vi "Initialize.vi"(8 "error in (no error)":errorcluster, 10 "Info":T1, 11 "Image in":refnum<class "SVGImage.lvclass">) -> (0 "error out":errorcluster, 3 "Image out":refnum<class "SVGImage.lvclass">)   [LabVIEW 2019, in "SVGImage.lvclass"]
uses:
  SVGImage.lvclass
  C:/Users/Albro/Documents/GitHub/AFM-Lithography/lvsrc/Classes/Parse/SVG Object/SVG Object.lvclass
  InitializationInfo.ctl
  TransformTokenizer/TransformTokenizer.lvclass
  TransformTokenizer/TransformTokenizer.lvclass/TransformTokenizer.ctl
  SVGImage.lvclass/SVGImage.ctl
  Transform/Transform.lvclass
  Transform.Matrix/Transform.Matrix.lvclass
  C:/Users/Albro/Documents/GitHub/AFM-Lithography/lvsrc/Classes/Parse/Transform/Transform.lvclass
  Transform.Translate/Transform.Translate.lvclass
  Transform.Rotate/Transform.Rotate.lvclass
  Transform.Skew/Transform.Skew.lvclass
  PathCommands/Point.ctl
  Transform/Transform.lvclass/Transform.ctl
  <vilib>/Analysis/baseanly.llb/Real A x B.vi
  Write X.vi
  Write Y.vi
  Write Width.vi
  Write Height.vi
  Write Path.vi
  Read Width.vi
  Read X.vi
  Read Height.vi
  Read Y.vi
  <vilib>/LabVIEW Open Source Project/OpenURI/openURI.lvlib
  PathCommands/PathCommands.lvclass
  <vilib>/Analysis/NI_AALBase.lvlib
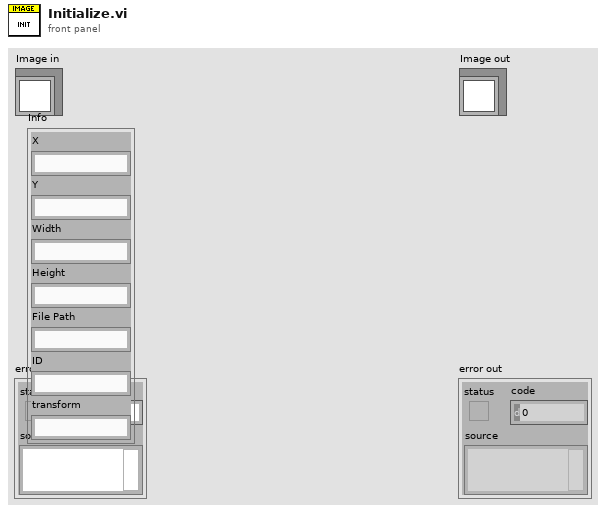
[diagram p1: front panel]
types:
  T1 = typedef "SVGImage.lvclass/InitializationInfo.ctl" = cluster{"X":string, "Y":string, "Width":string, "Height":string, "File Path":string, "ID":string, "transform":string}
  T2 = typedef "PathCommands.lvclass/Point.ctl" = cluster{"X":dbl, "Y":dbl}
  T3 = typedef "NI_Matrix.lvlib/RealMatrix.ctl" = dbl[][]
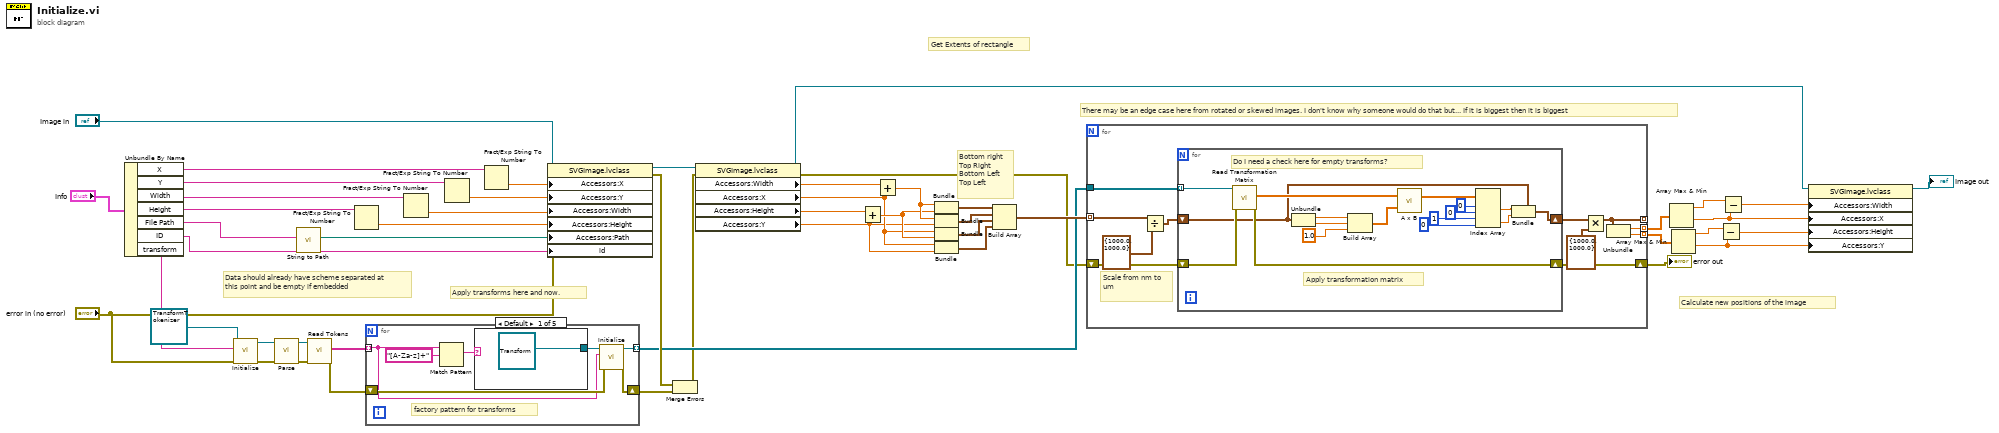
[diagram p0: block diagram]
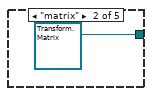
[diagram p2: hidden frame]
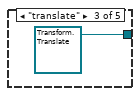
[diagram p3: hidden frame]
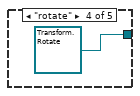
[diagram p4: hidden frame]
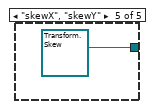
[diagram p5: hidden frame]
diagram:
  # "There may be an edge case here from rotated or skewed images. I don't know why someone would do that but... If it is biggest then it is biggest"
  # "Calculate new positions of the image"
  # "Get Extents of rectangle"
  # "Bottom right\nTop Right\nBottom Left\nTop Left"
  # "Apply transforms here and now."
  # "Data should already have scheme separated at this point and be empty if embedded"
  n1 = Unbundle By Name("Info") -> ("X"=w48:string, "Y"=w47:string, "Width"=w46:string, "Height"=w45:string, "File Path"=w39:string, "ID"=w38:string, "transform"=w1:string)
  n2 = call "Initialize.vi"("error in (no error)"="error in (no error)", "Transform Attribute String"=w1, "TransformTokenizer in"=refnum<class "TransformTokenizer.lvclass"> refnum) -> ("error out"=w37:errorcluster, "TransformTokenizer out"=w33:refnum<class "TransformTokenizer.lvclass">)  [unwired: 7 in]
  n3 = call "Parse.vi"("error in (no error)"=w37, "TransformTokenizer in"=w33) -> ("error out"=w36:errorcluster, "TransformTokenizer out"=w31:refnum<class "TransformTokenizer.lvclass">)  [unwired: 8 in]
  n4 = call <vilib>:"String to Path.vi"("common path"=w39) -> ("Path"=w40:path)  [unwired: 10 in]
  n5 = call "Read Tokens.vi"("error in (no error)"=w36, "TransformTokenizer in"=w31) -> ("error out"=w35:errorcluster, "Transforms"=w30:string[])  [unwired: 7 in, 1 out]
  n6 = Fract/Exp String To Number(string=w45) -> (number=w41:dbl)  [unwired: 3 in, 1 out]
  n7 = for {
    tunnel: w30 -> [w51] mode=indexing
    shift-right: [w53] -> w34
    shift-left: w35 -> [w54]
    tunnel: [w52] -> w15 mode=indexing
    # "factory pattern for transforms"
    n8 = Match Pattern(string=w51, regular expression="[A-Za-z]+") -> (match substring=w56:string)  [unwired: 1 in, 3 out]
    n9 = case shown="Default" w56 {
      tunnel: [refnum<class "Transform.lvclass"> refnum ("Transform in") refnum<class "Transform.Matrix.lvclass"> refnum ("Transform.Matrix.lvclass") refnum<class "Transform.Translate.lvclass"> refnum ("Transform.Translate.lvclass") refnum<class "Transform.Rotate.lvclass"> refnum ("Transform.Rotate.lvclass") refnum<class "Transform.Skew.lvclass"> refnum ("Transform.Skew.lvclass")] -> w55
      frame Default {
      }
      frame "matrix" {
      }
      frame "translate" {
      }
      frame "rotate" {
      }
      frame "skewX", "skewY" {
      }
    }
    n10 = call-dynamic "Initialize.vi"("error in (no error)"=w54, "Transform"=w51, "Transform in"=w55) -> ("error out"=w53:errorcluster, "Transform out"=w52:refnum<class "Transform.lvclass">)  [unwired: 7 in]
  }
  n11 = Fract/Exp String To Number(string=w46) -> (number=w42:dbl)  [unwired: 3 in, 1 out]
  n12 = Fract/Exp String To Number(string=w47) -> (number=w43:dbl)  [unwired: 3 in, 1 out]
  n13 = Fract/Exp String To Number(string=w48) -> (number=w44:dbl)  [unwired: 3 in, 1 out]
  n14 = property class="SVGImage.lvclass"(reference="Image in", error in="error in (no error)", "Accessors:X"=w44, "Accessors:Y"=w43, "Accessors:Width"=w42, "Accessors:Height"=w41, "Accessors:Path"=w40, "id"=w38) -> (reference out=w21:refnum<class "SVGImage.lvclass">, error out=w16:errorcluster)
  n15 = Merge Errors(w16, w34) -> (w13:errorcluster)
  n16 = property class="SVGImage.lvclass"(reference=w21, error in=w13) -> (reference out=w10:refnum<class "SVGImage.lvclass">, error out=w12:errorcluster, "Accessors:Width"=w20:dbl, "Accessors:X"=w19:dbl, "Accessors:Height"=w18:dbl, "Accessors:Y"=w17:dbl)
  n17 = Add(x=w18, y=w17) -> (x+y=w27:dbl)
  n18 = Add(x=w20, y=w19) -> (x+y=w28:dbl)
  n19 = Bundle(w28, w27) -> (w26:cluster{dbl, dbl})  [unwired: 1 in]
  n20 = Bundle(w28, "Accessors:Y"=w17) -> (w23:cluster{dbl, "Accessors:Y":dbl})  [unwired: 1 in]
  n21 = Bundle("Accessors:X"=w19, w27) -> (w25:cluster{"Accessors:X":dbl, dbl})  [unwired: 1 in]
  n22 = Bundle("Accessors:X"=w19, "Accessors:Y"=w17) -> (w24:cluster{"Accessors:X":dbl, "Accessors:Y":dbl})  [unwired: 1 in]
  n23 = Build Array(w26, w23, w25, w24) -> (w22:cluster{"Accessors:X":dbl, "Accessors:Y":dbl}[])
  n24 = for {
    tunnel: w15 -> [w73]
    shift-right: [w69] -> w14
    shift-left: w12 -> [w72]
    tunnel: w22 -> [w68] mode=indexing
    tunnel: [w64] -> _ mode=indexing
    tunnel: [w66] -> w9 mode=indexing
    tunnel: [w65] -> w6 mode=indexing
    # "Scale from nm to um"
    n25 = Divide(x=w68, y=T2 {"X"=1000.0, "Y"=1000.0} ("Point")) -> (x/y=w70:T2)
    n26 = for {
      tunnel: w73 -> [w90] mode=indexing
      shift-right: [w74] -> w67
      shift-left: w70 -> [w86]
      shift-right: [w87] -> w69
      shift-left: w72 -> [w88]
      # "Apply transformation matrix"
      # "Do I need a check here for empty transforms?"
      n27 = call "Read Transformation Matrix.vi"("error in (no error)"=w88, "Transform in"=w90) -> ("error out"=w87:errorcluster, "Real Matrix"=w89:T3)  [unwired: 7 in, 1 out]
      n28 = Unbundle(w86) -> ("X"=w85:dbl, "Y"=w84:dbl)
      n29 = Build Array(w85, w84, 1.0) -> (w75:T3)
      n30 = call-poly <vilib>:"A x B.vi"("B"=w75, "A"=w89) -> ("A x B"=w83:T3)  [unwired: 1 out]
      n31 = Index Array(array=w83, index (row) #1=0 ("index (row)"), index (col) #1=0 ("index (col)"), index (row) #2=1 ("index (row)"), index (col) #2=0 ("index (col)")) -> (element #1=w79:dbl, element #2=w78:dbl)
      n32 = Bundle(cluster=w86, "X"=w79, "Y"=w78) -> (w74:T2)
    }
    n33 = Multiply(x=w67, y=T2 {"X"=1000.0, "Y"=1000.0} ("Point")) -> (x*y=w64:T2)
    n34 = Unbundle(w64) -> ("X"=w66:dbl, "Y"=w65:dbl)
  }
  "error out" <- w14
  n35 = Array Max & Min(array=w9) -> (max value=w8:dbl, min value=w2:dbl)  [unwired: 2 out]
  n36 = Array Max & Min(array=w6) -> (max value=w5:dbl, min value=w3:dbl)  [unwired: 2 out]
  n37 = Subtract(x=w5, y=w3) -> (x-y=w4:dbl)
  n38 = Subtract(x=w8, y=w2) -> (x-y=w7:dbl)
  n39 = property class="SVGImage.lvclass"(reference=w10, "Accessors:Width"=w7, "Accessors:X"=w2, "Accessors:Height"=w4, "Accessors:Y"=w3) -> (reference out=→"Image out":refnum<class "SVGImage.lvclass">)  [unwired: 1 in, 1 out]
